vi "[ex ce] Tank Parameters History.vi"() -> ()   [LabVIEW 2021]
doc: "<B>Varible Manager example</B>\n\nThis example demonstrates a use of variable histories and aliases. It consists of two top-level VIs (when you run this VI, both the VIs will be launched):\n\n1) <B>[ex ce] Tank Simulator.vi</B> simulates a tank with inlet and outlet pipes. It creates a variable context with some variables to store parameters of work. Every variable gets a history attached and an alias. When the VI writes a variable value, the variable history is automatically updated.\n\n2) <B>[ex ce] Tank Parameters History.vi</B> reads history of the variables written by the previous VI and displays it on graphs. To access the variables, this VI uses their known aliases. This method makes it possible to access variables without a need to know a variable context where the variables reside.\n\n::: CalcExpress Toolkit :::\nCopyright (c) 2000-2026 Konstantin Shifershteyn. All rights reserved."
panel:
  out "History Graph":cluster{"time stamps":dbl[], "history":dbl[]}[](graph)
  in  "pause":bool
  in  "Display Timeframe, sec":dbl=60.0 min=10.0 max=300.0
  in  "Display offset, sec":dbl(slide) min=0.0 max=240.0 step=1.0
  in  "stop":bool
  # "This example consists of two top-level VIs:\n  [ex ce] Tank Simulator.vi  and\n  [ex ce] Tank Parameters History.vi\nWhen you run this VI, both the VIs will be launched."
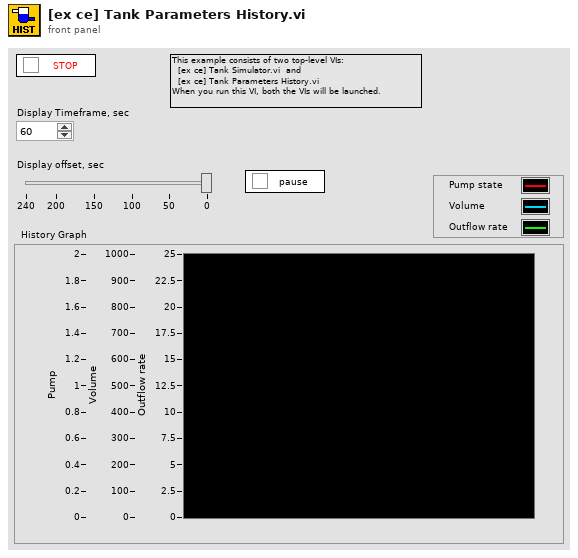
[diagram p1: front panel]
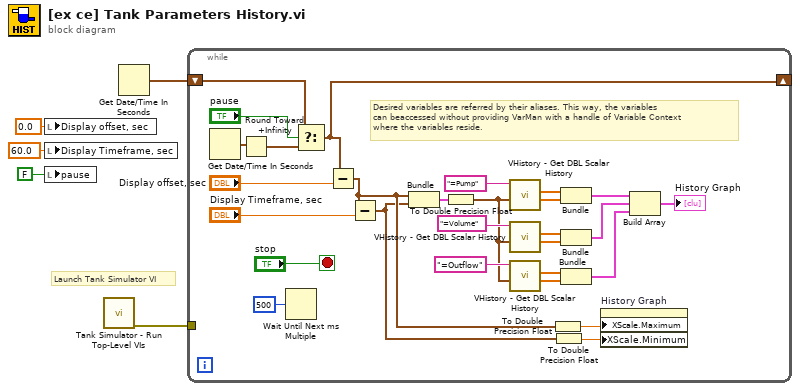
[diagram p0: block diagram]
diagram:
  # "Launch Tank Simulator VI"
  n1 = local write "Display offset, sec"(0.0 ("window offset, sec")) -> ()
  n2 = local write "Display Timeframe, sec"(60.0 ("window length, sec")) -> ()
  n3 = local write "pause"(FALSE ("pause")) -> ()
  n4 = call "Tank Simulator - Run Top-Level VIs.vi"() -> ("error out"=w2:errorcluster)  [unwired: 9 in]
  n5 = Get Date/Time In Seconds() -> (seconds since 1Jan1904=w1:timestamp)
  n6 = while {
    tunnel: w2 -> [_]
    shift-left: w1 -> [w28]
    shift-right: [w27] -> _
    stop <- "stop" stop-if-true
    # "Desired variables are referred by their aliases. This way, the variables\ncan beaccessed without providing VarMan with a handle of Variable Context\nwhere the variables reside."
    n7 = Get Date/Time In Seconds() -> (seconds since 1Jan1904=w9:timestamp)
    n8 = Round Toward +Infinity(x=w9) -> (ceil(x): smallest int >= x=w30:timestamp)
    n9 = Wait Until Next ms Multiple(millisecond multiple=u32 500) -> ()  [unwired: 1 out]
    n10 = Select(t=w28, s="pause", f=w30) -> (s? t:f=w27:timestamp)
    n11 = Subtract(x=w27, y="Display offset, sec") -> (x-y=w15:timestamp)
    n12 = Subtract(x=w15, y="Display Timeframe, sec") -> (x-y=w14:timestamp)
    n13 = Bundle(w15, w14) -> (w17:cluster{timestamp, timestamp})  [unwired: 1 in]
    n14 = To Double Precision Float(number=w17) -> (double precision float=w8:cluster{dbl, dbl})
    n15 = call "VHistory - Get DBL Scalar History.vi"("time range (all)"=w8, "name_spec"="=Pump" ("var name")) -> ("history"=w19:dbl[], "time stamps"=w18:dbl[])  [unwired: 5 in, 3 out]
    n16 = call "VHistory - Get DBL Scalar History.vi"("time range (all)"=w8, "name_spec"="=Volume" ("var name")) -> ("history"=w24:dbl[], "time stamps"=w25:dbl[])  [unwired: 5 in, 3 out]
    n17 = call "VHistory - Get DBL Scalar History.vi"("time range (all)"=w8, "name_spec"="=Outflow" ("var name")) -> ("history"=w22:dbl[], "time stamps"=w23:dbl[])  [unwired: 5 in, 3 out]
    n18 = To Double Precision Float(number=w15) -> (double precision float=w7:dbl)
    n19 = To Double Precision Float(number=w14) -> (double precision float=w6:dbl)
    n20 = Bundle("time stamps"=w18, "history"=w19) -> (w13:cluster{"time stamps":dbl[], "history":dbl[]})  [unwired: 1 in]
    n21 = Bundle("time stamps"=w25, "history"=w24) -> (w12:cluster{"time stamps":dbl[], "history":dbl[]})  [unwired: 1 in]
    n22 = Bundle("time stamps"=w23, "history"=w22) -> (w11:cluster{"time stamps":dbl[], "history":dbl[]})  [unwired: 1 in]
    n23 = property on="History Graph" class="XYGraph (strict)"("XScale.Maximum"=w7, "XScale.Minimum"=w6) -> ()  [unwired: 2 in, 2 out]
    n24 = Build Array(w13, w12, w11) -> (→"History Graph":cluster{"time stamps":dbl[], "history":dbl[]}[])
  }
